vi "Initialize Reader Data.vi"(8 "error in (no error)":errorcluster, 11 "CIF_Iceoryx_BB in":refnum<class "CIF_Iceoryx_Chn_String.lvclass">) -> (0 "error out":errorcluster, 3 "CIF_Iceoryx_BB out":refnum<class "CIF_Iceoryx_Chn_String.lvclass">)   [LabVIEW 2021, in "CIF_Iceoryx_Chn_String.lvclass"]
uses:
  CIF_Iceoryx_Chn_String.lvclass
  CIF_Iceoryx_Chn_String.lvclass/CIF_Iceoryx_Chn_String.ctl
  CIF_Iceoryx_BB/CIF_Iceoryx_BB.lvclass
  554698fa-34d1-4910-91f3-150097903222.vi
  D:/dev/Packages/CIF_Channels_Core/src/Iceorxy_Channels/CIF_Iceoryx_BB/CIF_Iceoryx_BB.lvclass
  D:/dev/Packages/CIF_Channels_Core/src/Iceorxy_Channels/CIF_Iceoryx_Chan/CIF_Iceoryx_Chn.lvclass
  D:/dev/Packages/CIF_Channels_Core/src/CIFChannels/CIFChannels.lvclass
  D:/dev/Packages/CIF_Channels_Core/src/Iceorxy_Channels/String/CIF_Iceoryx_Chn_String.lvclass
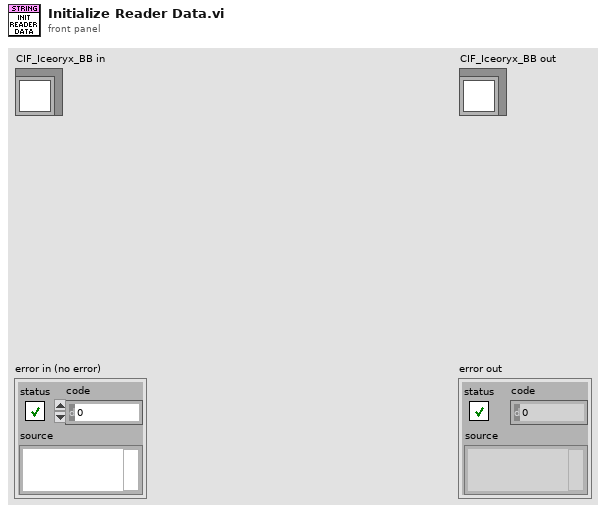
[diagram p1: front panel]
types:
  T1 = typedef "Iceoryx.lvlib/BB Reader Refnum.ctl" = cluster{"refnum":u64, "BB Reader":enum8{"bb_reader"}}
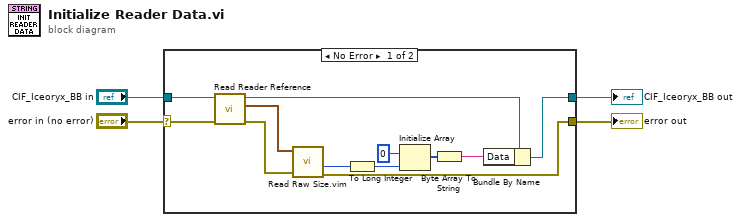
[diagram p0: block diagram]
diagram:
  n1 = case shown="No Error" "error in (no error)" {
    selector: "error in (no error)" -> [w15 w18]
    tunnel: "CIF_Iceoryx_BB in" -> [w16 w17]
    tunnel: [w6 w17] -> w3
    tunnel: [w5 w18] -> w1
    frame No Error {
      n2 = call "Read Reader Reference.vi"("error in (no error)"=w15, "CIF_Iceoryx_BB in"=w16) -> ("error out"=w13:errorcluster, "BB Reader Refnum"=w14:T1, "CIF_Iceoryx_BB out"=w9:refnum<class "CIF_Iceoryx_Chn_String.lvclass">)  [unwired: 7 in]
      n3 = call "Read Raw Size.vim"("error in (no error)"=w13, "Raw Reader Reference"=w14) -> ("error out"=w5:errorcluster, "Max Bytes"=w10:u32)  [unwired: 8 in]
      n4 = To Long Integer(number=w10) -> (32bit integer=w11:i32)
      n5 = Initialize Array(u8 0 ("Buffer Size N (2^N)"), w11) -> (w8:u8[])
      n6 = Byte Array To String(unsigned byte array=w8) -> (string=w7:string)
      n7 = Bundle By Name(cluster=w9, "Data"=w7) -> (w6:refnum<class "CIF_Iceoryx_Chn_String.lvclass">)
    }
    frame Error {
    }
  }
  "error out" <- w1
  "CIF_Iceoryx_BB out" <- w3
